vi "DAQmx.AI Max to Range.vi"(11 "AI.Max":dbl) -> (3 "Range":T1)   [LabVIEW 2019, in "DAQmx.lvclass"]
uses:
  DAQmx.lvclass
  typedefs/DAQmx.Config.AI.Range--enum.ctl
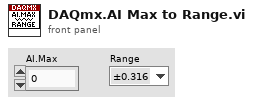
[diagram p1: front panel]
types:
  T1 = typedef "DAQmx.lvclass/DAQmx.Config.AI.Range--enum.ctl" = enum16{"±0.316", "±1.00", "±3.16", "±10.0", "±31.6", "±42.4"}
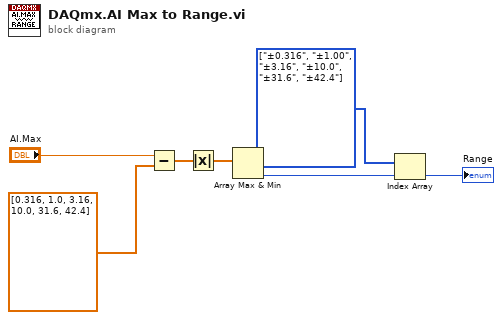
[diagram p0: block diagram]
diagram:
  w3 = T1[] [enum."±0.316", enum."±1.00", enum."±3.16", enum."±10.0", enum."±31.6", enum."±42.4"] items=["±0.316", "±1.00", "±3.16", "±10.0", "±31.6", "±42.4"] ("Range")
  n1 = Subtract(x="AI.Max", y=dbl[] [0.316, 1.0, 3.16, 10.0, 31.6, 42.4]) -> (x-y=w5:dbl[])
  n2 = Absolute Value(x=w5) -> (abs(x)=w4:dbl[])
  n3 = Array Max & Min(array=w4) -> (min index (indices)=w2:i32)  [unwired: 3 out]
  n4 = Index Array(array=w3, index=w2) -> (element=→"Range":T1)
